vi "Sort out Display from State.vi"(4 "Func In":refnum<vi>, 6 "Starting Phase In":refnum<vi>, 7 "Data In":T1, 8 "Error In (no Error) In":errorcluster, 9 "Display In":refnum<vi>, 10 "Controls In":refnum<vi>, 11 "Display State In":T2={"Show Axes"=FALSE, "Show Y=0"=FALSE, "Controls"={"Type"=enum."Sine", "Periods"=0.0, "Points"=0, "Offset"=0.0, "Amplitdue"=0.0, "Phase"=0.0, "func"=""}, "Show Current Location"=FALSE, "Current Location"=0, "dt"=0.0, "t0"=timestamp(0 s since 1904-01-01), "Format and Units"="%_3p"} caption="State") -> (0 "Error Out":errorcluster, 3 "Display State Out":T2={"Show Axes"=FALSE, "Show Y=0"=FALSE, "Controls"={"Type"=enum."Sine", "Periods"=0.0, "Points"=0, "Offset"=0.0, "Amplitdue"=0.0, "Phase"=0.0, "func"=""}, "Show Current Location"=FALSE, "Current Location"=0, "dt"=0.0, "t0"=timestamp(0 s since 1904-01-01), "Format and Units"="%_3p"} caption="State")   [LabVIEW 2012, in "Waveform Control.xctl"]
doc: "Formats the display of the XControl according to the state"
uses:
  Waveform Control.xctl
  Controls/Waveform State.ctl
  FP Controls.ctl
  Function Types.ctl
  Controls/Data.ctl
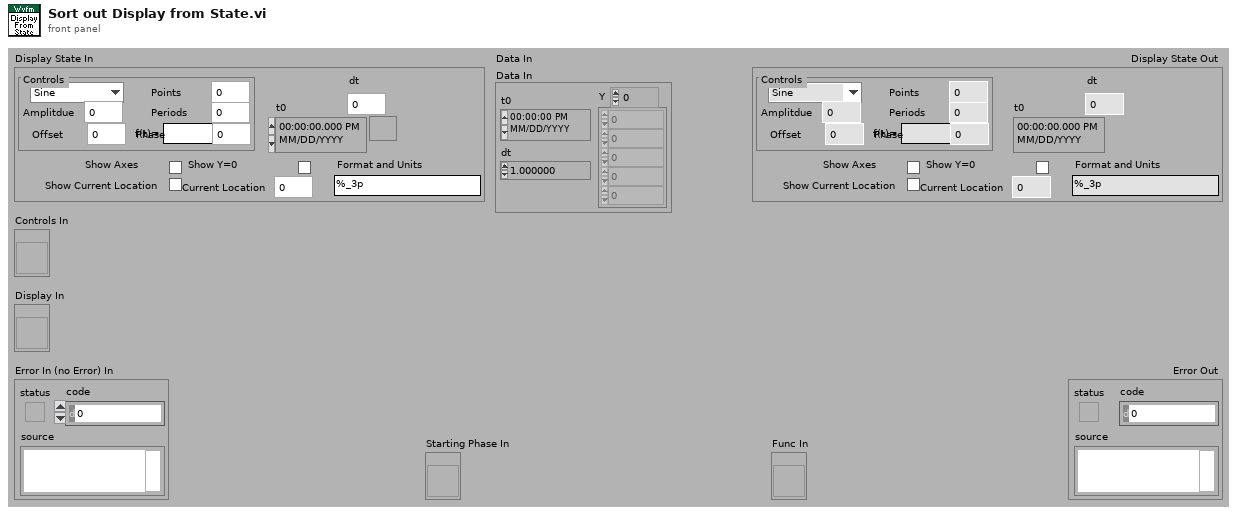
[diagram p1: front panel]
types:
  T1 = typedef "Waveform Control.xctl/Data.ctl" = waveform(dbl)
  T2 = typedef "Waveform Control.xctl/Waveform State.ctl" = cluster{"Show Axes":bool, "Show Y=0":bool, "Controls":T3, "Show Current Location":bool, "Current Location":i32, "dt":dbl, "t0":timestamp, "Format and Units":string}
  T3 = typedef "Waveform Control.xctl/FP Controls.ctl" = cluster{"Type":T4, "Periods":dbl, "Points":i32, "Offset":dbl, "Amplitdue":dbl, "Phase":dbl, "func":string}
  T4 = typedef "Waveform Control.xctl/Function Types.ctl" = enum16{"Level", "Sine", "Triangle", "Ramp", "Saw Tooth", "Square", "Function"}
  T5 = cluster{"Show Axes":bool, "Show Y=0":bool, "Controls":cluster{"Type":bool, "Periods":bool, "Points":bool, "Offset":bool, "Amplitdue":bool, "Phase":bool, "func":bool}, "Show Current Location":bool, "Current Location":bool, "dt":bool, "t0":bool, "Format and Units":bool}
  T6 = cluster{"Type":bool, "Periods":bool, "Points":bool, "Offset":bool, "Amplitdue":bool, "Phase":bool, "func":bool}
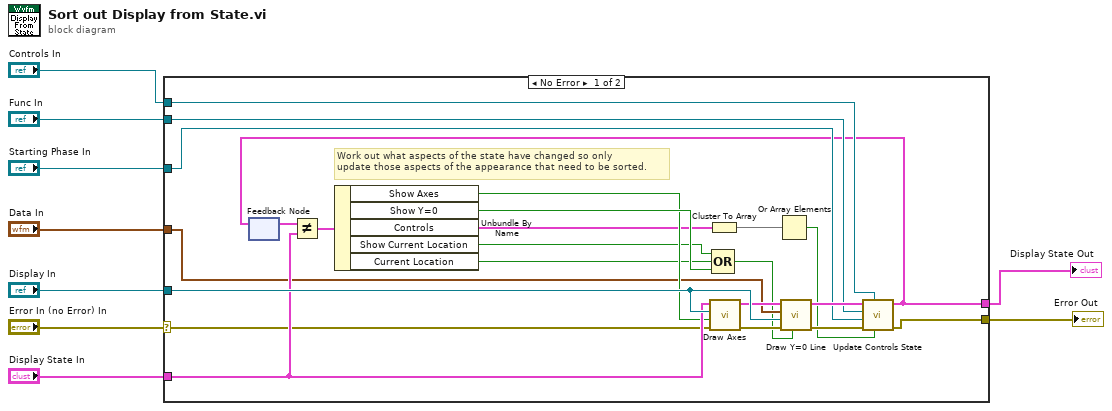
[diagram p0: block diagram]
diagram:
  n1 = case shown="No Error" "Error In (no Error) In" {
    selector: "Error In (no Error) In" -> [w28 w34]
    tunnel: "Display In" -> [w31 _]
    tunnel: "Display State In" -> [w29 w33]
    tunnel: "Starting Phase In" -> [w24 _]
    tunnel: "Func In" -> [w23 _]
    tunnel: "Controls In" -> [w22 _]
    tunnel: [w10 w34] -> w4
    tunnel: [w13 w33] -> w3
    tunnel: "Data In" -> [w15 _]
    frame No Error {
      # "Work out what aspects of the state have changed so only\nupdate those aspects of the appearance that need to be sorted."
      n2 = feedback #1() -> (w14:T2)  [unwired: 1 out]
      n3 = Not Equal?(x=w14, y=w29) -> (x != y?=w16:T5)
      n4 = Unbundle By Name(w16) -> ("Show Axes"=w21:bool, "Show Y=0"=w32:bool, "Controls"=w19:T6, "Show Current Location"=w18:bool, "Current Location"=w17:bool)
      n5 = Cluster To Array(cluster=w19) -> (array=w20:bool[])
      n6 = call "Draw Axes.vi"("Error In (no Error) In"=w28, "Show Axes In"=w21, "WFGraph Refnum In"=w31, "Display State In"=w29) -> ("Error Out"=w27:errorcluster, "Display State Out"=w30:T2)  [unwired: 6 out]
      n7 = Compound Arithmetic op=OR(w18, w17, w32) -> (w12:bool)
      n8 = Or Array Elements(Boolean array=w20) -> (logical OR=w11:bool)
      n9 = call "Draw Y=0 Line.vi"("Needs Update In"=w12, "Error In (no Error) In"=w27, "PreviewGraph Ref In"=w31, "Data In"=w15, "Display State In"=w30) -> ("Error Ou Out"=w26:errorcluster, "Display State Out"=w25:T2)  [unwired: 2 in, 3 out]
      n10 = call "Update Controls State.vi"("Controls Need Update In"=w11, "Controlst In"=w22, "Error In (no Error) In"=w26, "DigNum Refnum In"=w24, "Str Refnum In"=w23, "Display State In"=w25) -> ("Error Out"=w10:errorcluster, "Display State Out"=w13:T2)  [unwired: 4 out]
      n11 = feedback-in #1(w13) -> ()
    }
    frame Error {
    }
  }
  "Error Out" <- w4
  "Display State Out" <- w3
